vi "set Sweep Time.vi"(8 "error in (no error)":errorcluster, 9 "Sweep Time Auto?":bool, 10 "Sweep Time(sec)":dbl, 11 "FSV-40N in":refnum<class "FSV-40N.lvclass">) -> (0 "error out":errorcluster, 3 "FSV-40N out":refnum<class "FSV-40N.lvclass">)   [LabVIEW 2023, in "Spectrum Analyzer.lvlib" / "FSV-40N.lvclass"]
uses:
  FSV-40N.lvclass
  FSV-40N.lvclass/FSV-40N.ctl
  <vilib>/ErrorRing/Error Ring.xnode
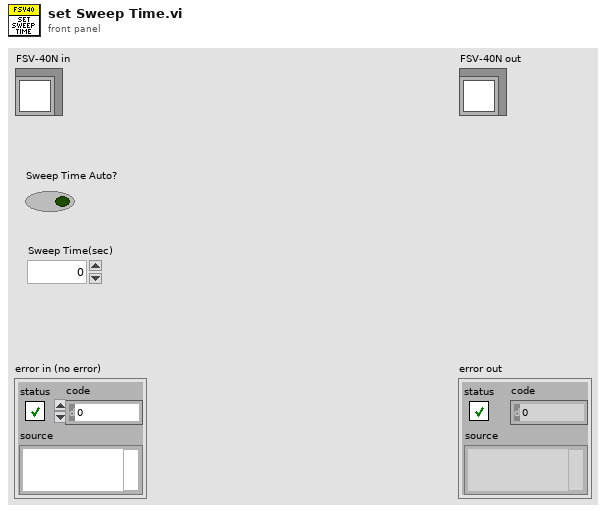
[diagram p1: front panel]
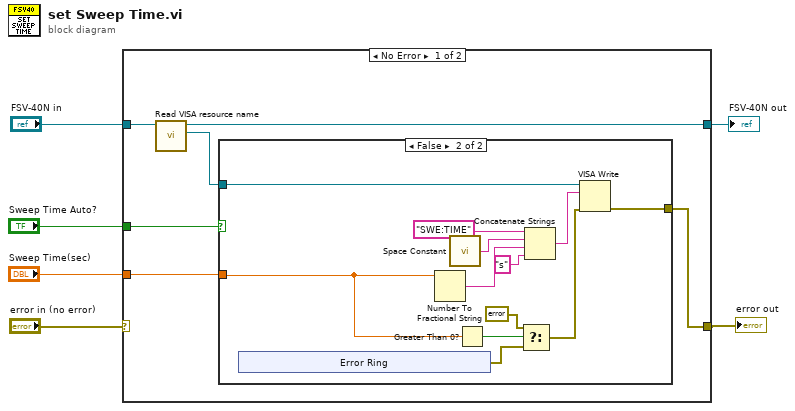
[diagram p0: block diagram]
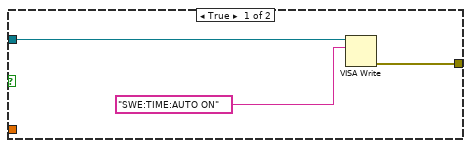
[diagram p2: hidden frame]
diagram:
  n1 = case shown="No Error" "error in (no error)" {
    selector: "error in (no error)" -> [_ w29]
    tunnel: "FSV-40N in" -> [w12 w30]
    tunnel: [w10 w30] -> w5
    tunnel: [w7 w29] -> w3
    tunnel: "Sweep Time Auto?" -> [w11 _]
    tunnel: "Sweep Time(sec)" -> [w8 _]
    frame No Error {
      n2 = call "Read VISA resource name.vi"("FSV-40N in"=w12) -> ("VISA resource name"=w9:refnum<visa-resource-name>, "FSV-40N out"=w10:refnum<class "FSV-40N.lvclass">)  [unwired: 8 in, 1 out]
      n3 = case shown="False" w11 {
        tunnel: w9 -> [w15 w27]
        tunnel: [w13 w26] -> w7
        tunnel: w8 -> [_ w20]
        frame True {
          n4 = VISA Write(VISA resource name=w15, write buffer="SWE:TIME:AUTO ON") -> (error out=w13:errorcluster)  [unwired: 1 in, 2 out]
        }
        frame False {
          n5 = xnode "Error Ring"() -> ("error out"=w17:errorcluster)
          n6 = Number To Fractional String(number=w20) -> (F-format string=w23:string)  [unwired: 3 in]
          n7 = call <vilib>:"Space Constant.vi"() -> ("String"=w24:string)
          n8 = Greater Than 0?(x=w20) -> (x > 0?=w19:bool)
          n9 = Select(t=errorcluster {"status"=FALSE, "code"=0, "source"=""} ("error constant"), s=w19, f=w17) -> (s? t:f=w16:errorcluster)
          n10 = Concatenate Strings("SWE:TIME" ("write buffer"), w24, w23, "s" ("string")) -> (w21:string)
          n11 = VISA Write(VISA resource name=w27, write buffer=w21, error in (no error)=w16) -> (error out=w26:errorcluster)  [unwired: 2 out]
        }
      }
    }
    frame Error {
    }
  }
  "error out" <- w3
  "FSV-40N out" <- w5
